vi "Handle_Cmd.vi"(6 "folder ready":path, 8 "error in":errorcluster, 9 "timed out?":bool, 10 "data IN":T1, 11 "FPGA VI Reference IN":refnum<k20>) -> (0 "error out":errorcluster, 3 "FPGA VI Reference out":refnum<k20>)   [LabVIEW 2025]
uses:
  RT_Cmd.ctl
  Command.ctl
  vi/thresholds.ctl
  <vilib>/rvi/interface/nirviReadWriteControl/nirviReadWriteControl.xnode
  <vilib>/rvi/interface/nirviMethod/nirviMethod.xnode
  NiFpgaLv.dll
  <vilib>/Utility/error.llb/Error Cluster From Error Code.vi
  <vilib>/rvi/interface/Simulation/niFpgaSimulationCallBeginRW.vi
  <vilib>/rvi/errors/niLvFpgaAdjustHostInterfaceError.vi
  <vilib>/FPGAPlugInAG/Dynamic/niLvFpga_WriteFifo_Dynamic.vi
  <vilib>/rvi/errors/niLvFpgaMergeErrorWithErrorCode.vi
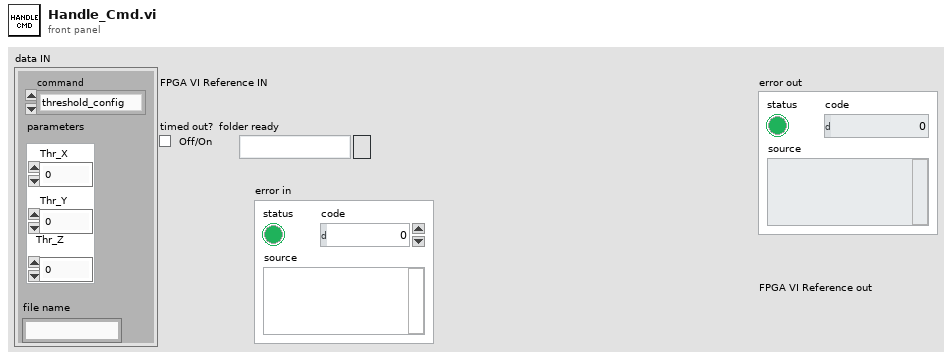
[diagram p1: front panel]
types:
  T1 = typedef "RT_Cmd.ctl" = cluster{"command":T2, "parameters":T3, "file name":string}
  T2 = typedef "Command.ctl" = enum16{"threshold_config", "manual_trigger", "stop", "remove_file"}
  T3 = typedef "thresholds.ctl" = cluster{"Thr_X":i16, "Thr_Y":i16, "Thr_Z":i16}
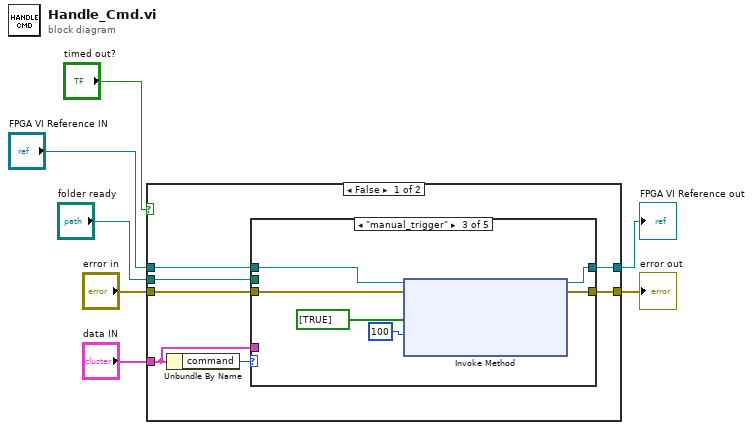
[diagram p0: block diagram]
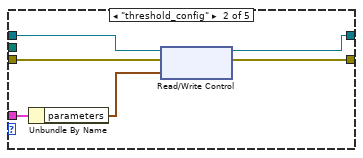
[diagram p3: hidden frame]
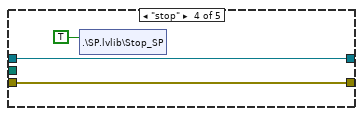
[diagram p4: hidden frame]
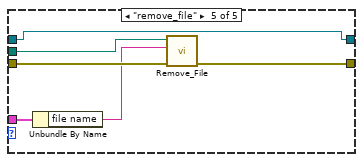
[diagram p5: hidden frame]
diagram:
  n1 = case shown="False" "timed out?" {
    tunnel: "data IN" -> [w13 _]
    tunnel: "FPGA VI Reference IN" -> [w12 w39]
    tunnel: [w11 w39] -> w1
    tunnel: "error in" -> [w10 w38]
    tunnel: [w9 w38] -> w3
    tunnel: "folder ready" -> [w8 _]
    frame False {
      n2 = Unbundle By Name(w13) -> ("command"=w14:T2)
      n3 = case shown="\"manual_trigger\"" w14 {
        tunnel: w13 -> [_ w22 _ _ w37]
        tunnel: w12 -> [w15 w21 w28 w30 w32]
        tunnel: [w15 w19 w23 w30 w32] -> w11
        tunnel: w10 -> [w16 w18 w25 w29 w36]
        tunnel: [w16 w17 w24 w29 w33] -> w9
        tunnel: w8 -> [_ _ _ _ w34]
        frame Default {
        }
        frame "threshold_config" {
          n4 = Unbundle By Name(w22) -> ("parameters"=w20:T3)
          n5 = xnode "Read/Write Control"("FPGA VI Reference In"=w21, "error in"=w18, "Threshold"=w20) -> ("FPGA VI Reference Out"=w19:refnum<k20>, "error out"=w17:errorcluster)
        }
        frame "manual_trigger" {
          n6 = xnode "Invoke Method"("FPGA VI Reference In"=w28, "error in"=w25, "Data"=bool[] [TRUE], "Timeout (ms)"=100) -> ("FPGA VI Reference Out"=w23:refnum<k20>, "error out"=w24:errorcluster)  [unwired: 1 out]
        }
        frame "stop" {
          n7 = shared-variable ".\\SP.lvlib\\Stop_SP"(TRUE ("Stop_SP")) -> ()  [unwired: 1 in, 1 out]
        }
        frame "remove_file" {
          n8 = Unbundle By Name(w37) -> ("file name"=w35:string)
          n9 = call "Remove_File.vi"("error in"=w36, "file name"=w35, "folder ready"=w34) -> ("error out"=w33:errorcluster)  [unwired: 8 in]
        }
      }
    }
    frame True {
    }
  }
  "error out" <- w3
  "FPGA VI Reference out" <- w1
